vi "temporary load classes.vi"(8 "error in":errorcluster, 10 "Config Class Path":path, 11 "Runtime Class Path":path) -> (0 "error out":errorcluster, 1 "Index Ctl":string[](array[string]), 2 "Data Ctl":string[](array[string]), 3 "valid?":bool[](array[boolean]), 4 "Channel Types":T1[](array[typedef]), 5 "Classifications":T1[](array[typedef])=[enum."input data", enum."output data", enum."processing parameter", enum."processing result"])   [LabVIEW 2014, in "control module data interface generator.lvlib"]
uses:
  control module data interface generator.lvlib
  <vilib>/NI/Tag Bus Module Framework/channel/channel classification.ctl
  configuration/control module configuration.lvclass
  runtime/control module runtime.lvclass
  <vilib>/Utility/VariantDataType/VariantType.lvlib
  <vilib>/NI/Tag Bus Module Framework/channel/TBM channel.lvclass
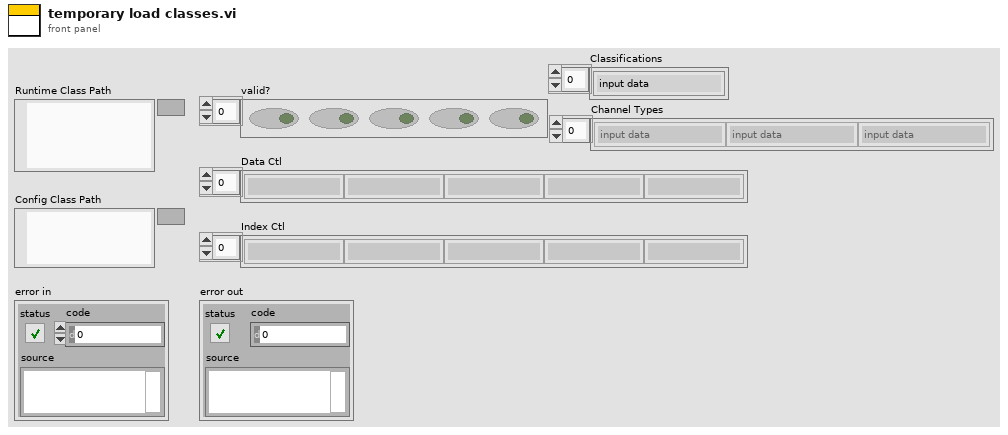
[diagram p1: front panel]
types:
  T1 = typedef "TBM channel.lvclass/channel classification.ctl" = enum16{"input data", "output data", "processing parameter", "processing result"}
  T2 = typedef "VariantType.lvlib/TypedefInfo.ctl" = cluster{"Name":string, "Timestamp":u32}
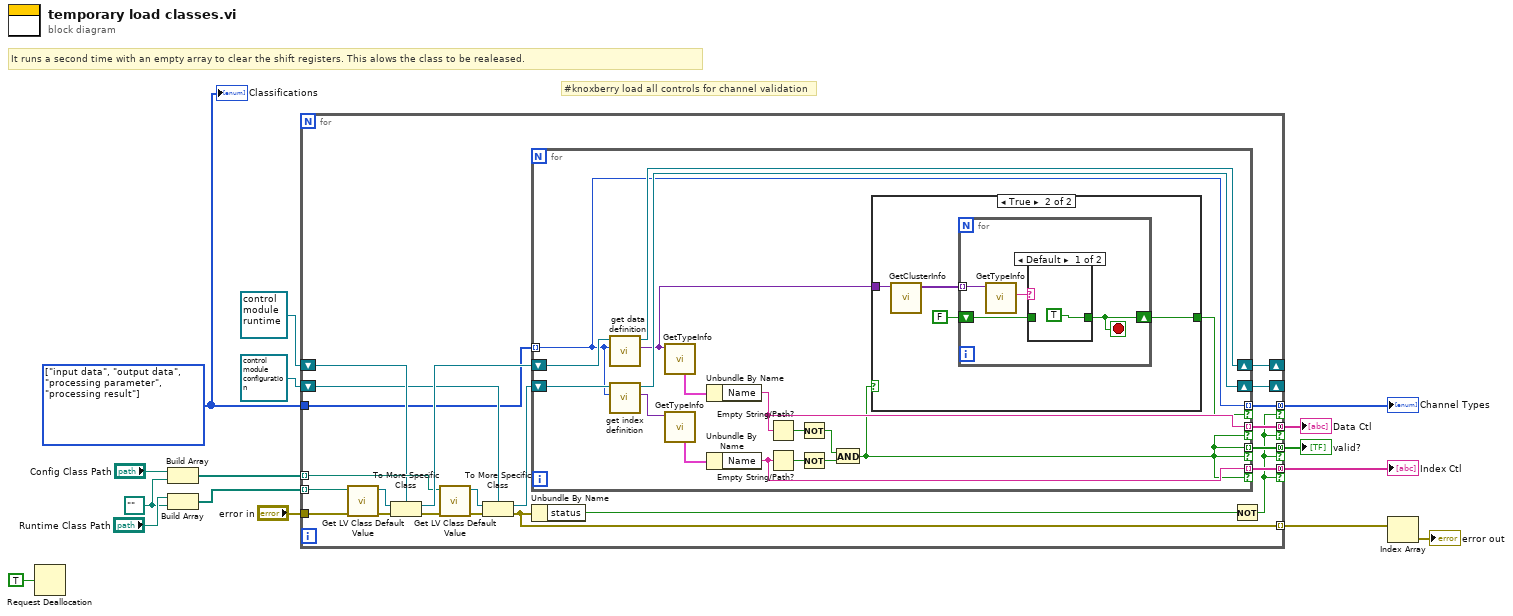
[diagram p0: block diagram]
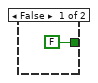
[diagram p2: hidden frame]
diagram:
  w2 = T1[] [enum."input data", enum."output data", enum."processing parameter", enum."processing result"] items=["input data", "output data", "processing parameter", "processing result"] ("classifications")
  w6 = path "" ("element")
  # "It runs a second time with an empty array to clear the shift registers. This alows the class to be realeased."
  # "#knoxberry load all controls for channel validation"
  n1 = Request Deallocation(TRUE ("flag")) -> ()
  n2 = Build Array("Config Class Path", w6) -> (w7:path[])
  n3 = Build Array("Runtime Class Path", w6) -> (w8:path[])
  n4 = for {
    tunnel: [w38] -> w16 mode=concatenating if=w17
    tunnel: [w37] -> w15 mode=concatenating if=w17
    tunnel: [w36] -> w14 mode=concatenating if=w17
    tunnel: w7 -> [w28] mode=indexing
    tunnel: w8 -> [w27] mode=indexing
    tunnel: "error in" -> [w35]
    tunnel: [w26] -> w12 mode=indexing
    shift-right: [w22] -> _
    shift-left: refnum<class "control module runtime.lvclass"> refnum ("fixed channel runtime") -> [w24]
    shift-right: [w20] -> _
    shift-left: refnum<class "control module configuration.lvclass"> refnum ("fixed channel configuration") -> [w23]
    tunnel: w2 -> [w19]
    tunnel: [w18] -> w1 mode=concatenating if=w17
    n5 = call <vilib>:"Get LV Class Default Value.vi"("error in (no error)"=w35, "class path"=w27) -> ("error out"=w32:errorcluster, "object"=w31:refnum<class>)  [unwired: 8 in]
    n6 = To More Specific Class(target class=w24, reference=w31, error in=w32) -> (specific class reference=w33:refnum<class "control module runtime.lvclass">, error out=w34:errorcluster)
    n7 = call <vilib>:"Get LV Class Default Value.vi"("error in (no error)"=w34, "class path"=w28) -> ("error out"=w29:errorcluster, "object"=w30:refnum<class>)  [unwired: 8 in]
    n8 = To More Specific Class(target class=w23, reference=w30, error in=w29) -> (specific class reference=w21:refnum<class "control module configuration.lvclass">, error out=w26:errorcluster)
    n9 = for {
      tunnel: [w40] -> w36 mode=indexing if=w40
      tunnel: [w54] -> w37 mode=indexing if=w40
      tunnel: [w53] -> w38 mode=indexing if=w40
      shift-right: [w50] -> w22
      shift-left: w33 -> [w51]
      shift-right: [w48] -> w20
      shift-left: w21 -> [w49]
      tunnel: w19 -> [w42] mode=indexing
      tunnel: [w42] -> w18 mode=indexing if=w39
      n10 = call-dynamic "get data definition.vi"("channel classification"=w42, "fixed channel runtime in"=w51) -> ("index cluster"=w41:variant, "fixed channel runtime out"=w50:refnum<class "control module runtime.lvclass">)  [unwired: 7 in, 1 out]
      n11 = call-dynamic "get index definition.vi"("channel classification"=w42, "fixed channel configuration in"=w49) -> ("index cluster"=w43:variant, "fixed channel configuration out"=w48:refnum<class "control module configuration.lvclass">)  [unwired: 7 in, 1 out]
      n12 = call <vilib>:"GetTypeInfo.vi"("Variant"=w41) -> ("TypedefInfo"=w45:T2)  [unwired: 6 in, 4 out]
      n13 = call <vilib>:"GetTypeInfo.vi"("Variant"=w43) -> ("TypedefInfo"=w46:T2)  [unwired: 6 in, 4 out]
      n14 = Unbundle By Name(w45) -> ("Name"=w54:string)
      n15 = Unbundle By Name(w46) -> ("Name"=w53:string)
      n16 = Empty String/Path?(string/path=w54) -> (empty?=w44:bool)
      n17 = Empty String/Path?(string/path=w53) -> (empty?=w47:bool)
      n18 = Not(x=w44) -> (.not. x?=w55:bool)
      n19 = Not(x=w47) -> (.not. x?=w52:bool)
      n20 = And(x=w55, y=w52) -> (x .and. y?=w40:bool)
      n21 = case shown="True" w40 {
        tunnel: [FALSE w58] -> w39
        tunnel: w41 -> [_ w57]
        frame False {
        }
        frame True {
          n22 = call <vilib>:"GetClusterInfo.vi"("Variant"=w57) -> ("Cluster Elements"=w60:variant[])  [unwired: 9 in, 1 out]
          n23 = for {
            tunnel: w60 -> [w64] mode=indexing
            shift-right: [w61] -> w58
            shift-left: FALSE -> [w62]
            stop <- w61 stop-if-true
            n24 = call <vilib>:"GetTypeInfo.vi"("Variant"=w64) -> ("Name"=w63:string)  [unwired: 6 in, 4 out]
            n25 = case shown="Default" w63 {
              tunnel: [TRUE w66] -> w61
              tunnel: w62 -> [_ w66]
              frame Default {
              }
              frame "", "fmwk_placeholder" {
              }
            }
          }
        }
      }
    }
    n26 = Unbundle By Name(w26) -> ("status"=w25:bool)
    n27 = Not(x=w25) -> (.not. x?=w17:bool)
  }
  "Index Ctl" <- w16
  "Data Ctl" <- w15
  "valid?" <- w14
  "Channel Types" <- w1
  n28 = Index Array(array=w12) -> (element=→"error out":errorcluster)  [unwired: 1 in]
  "Classifications" <- w2
